vi "Read Message.vi"(11 "LogMessage In":refnum<class "AbstractLogMessage.lvclass">) -> (2 "Message":string, 3 "LogMessage Out":refnum<class "AbstractLogMessage.lvclass">)   [LabVIEW 2020, in "AbstractLogMessage.lvclass"]
uses:
  AbstractLogMessage.lvclass
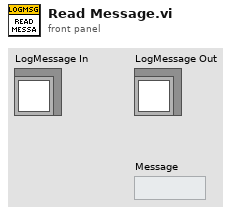
[diagram p1: front panel]
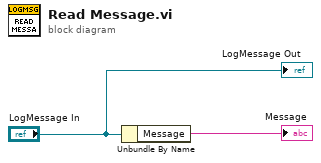
[diagram p0: block diagram]
diagram:
  n1 = Unbundle By Name("LogMessage In") -> ("Message"=→"Message":string)
  "LogMessage Out" <- "LogMessage In"
